vi "VF Laser Control.vi"(0 "Laser Notifier Element":T1={"Laser Action"=enum."Set On/Off", "Received?"=FALSE, "Enabled (Interlock)?"=FALSE, "Light Emission?"=FALSE, "Power (mW)"=0.0, "Settings"={"Laser Parameters"=enum."Wavelength (nm)", "Value"=0.0}, "Status"=enum."Error", "Error"={"status"=FALSE, "code"=0, "source"=""}}, 11 "VISA Ref":refnum<visa-resource-name>) -> (4 "Laser Notifier Element":T1={"Laser Action"=enum."Set On/Off", "Received?"=FALSE, "Enabled (Interlock)?"=FALSE, "Light Emission?"=FALSE, "Power (mW)"=0.0, "Settings"={"Laser Parameters"=enum."Wavelength (nm)", "Value"=0.0}, "Status"=enum."Error", "Error"={"status"=FALSE, "code"=0, "source"=""}})   [LabVIEW 2016]
uses:
  Laser Controls/Laser Notifier Element.ctl
  Laser Controls/Laser Actions.ctl
  Laser Controls/Laser Settings.ctl
  Laser Controls/Laser Parameters.ctl
  Laser Controls/Laser Status.ctl
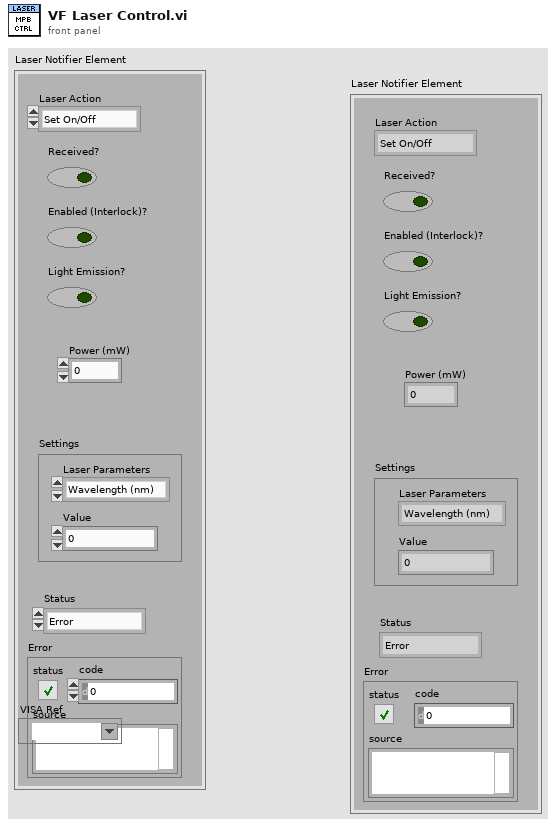
[diagram p1: front panel]
types:
  T1 = typedef "Laser Notifier Element.ctl" = cluster{"Laser Action":T2, "Received?":bool, "Enabled (Interlock)?":bool, "Light Emission?":bool, "Power (mW)":dbl, "Settings":T3, "Status":T5, "Error":errorcluster}
  T2 = typedef "Laser Actions.ctl" = enum16{"Error Check", "Set On/Off", "Set Power", "Set Parameter", "Get Power", "Get Status", "Get Parameter", "Quit"}
  T3 = typedef "Laser Settings.ctl" = cluster{"Laser Parameters":T4, "Value":dbl}
  T4 = typedef "Laser Parameters.ctl" = enum16{"Wavelength (nm)", "Pulsing?", "Rep. Rate"}
  T5 = typedef "Laser Status.ctl" = enum16{"Warmup", "Ready", "Emission", "Tuning", "Error"}
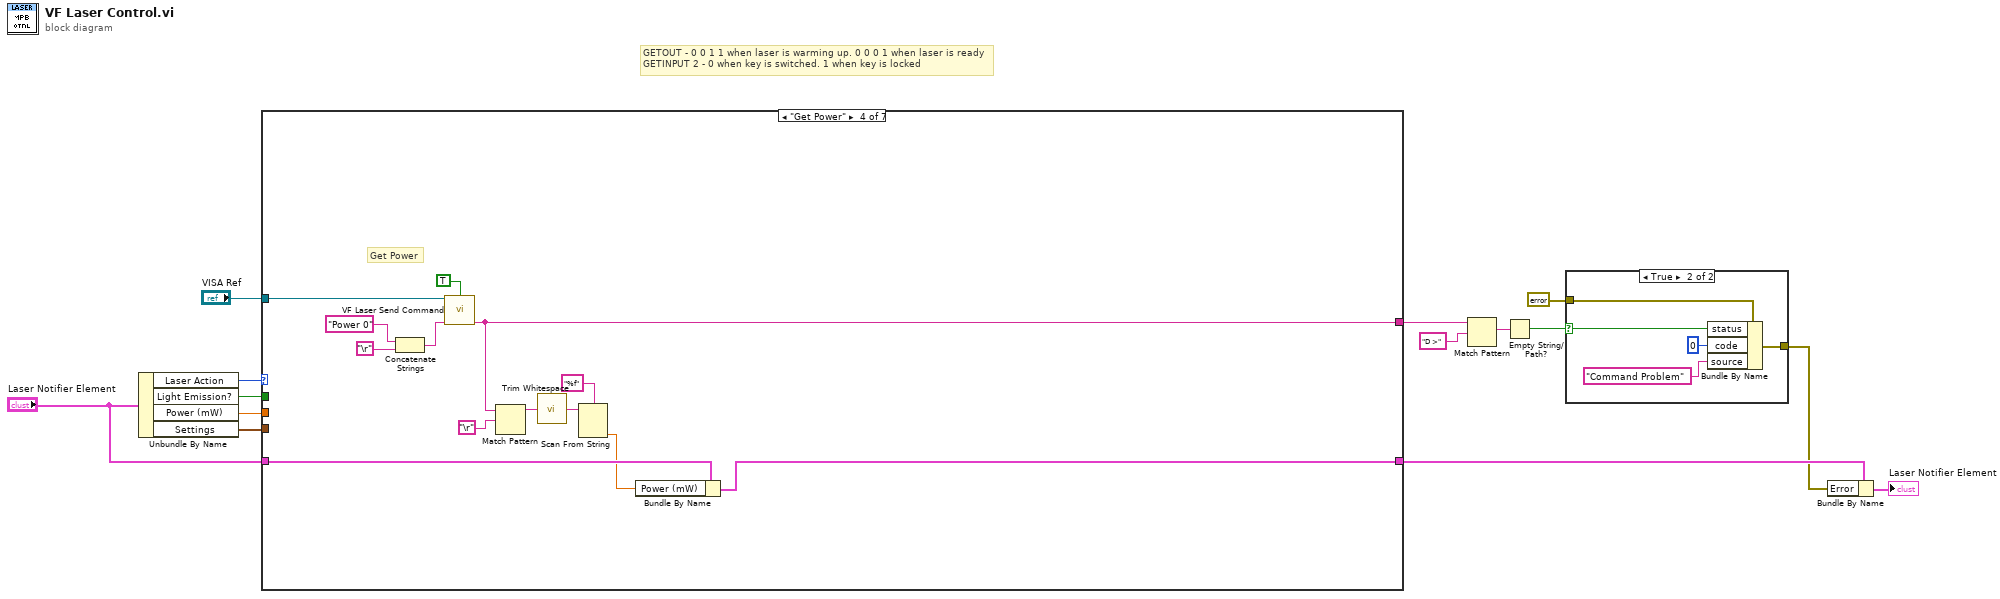
[diagram p0: block diagram]
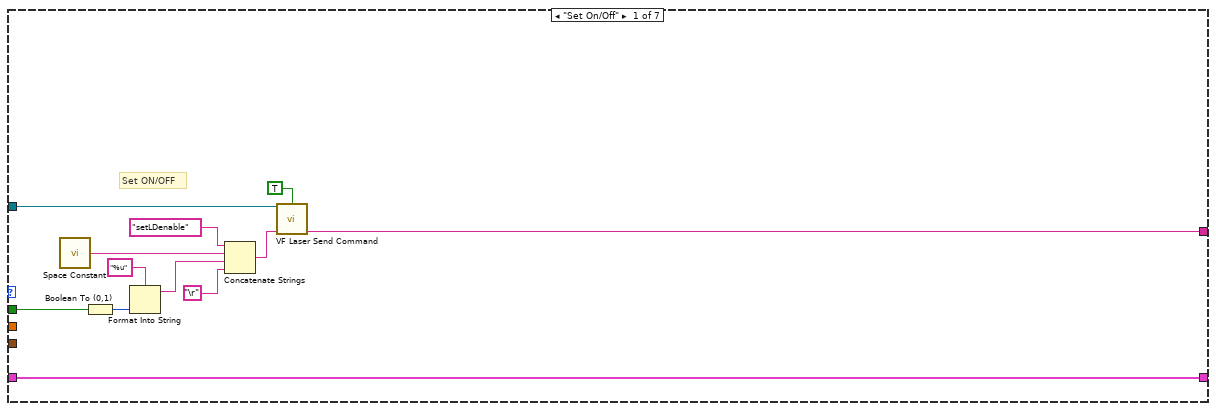
[diagram p3: hidden frame]
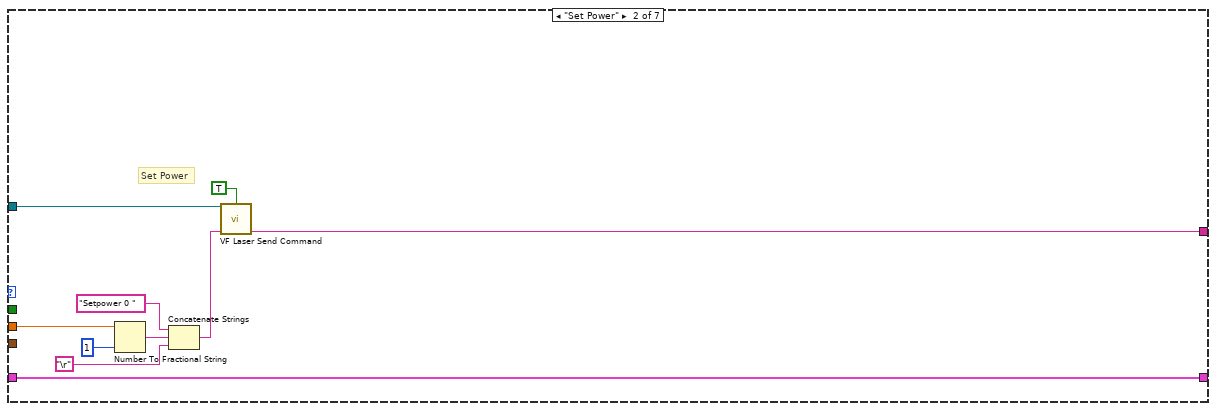
[diagram p4: hidden frame]
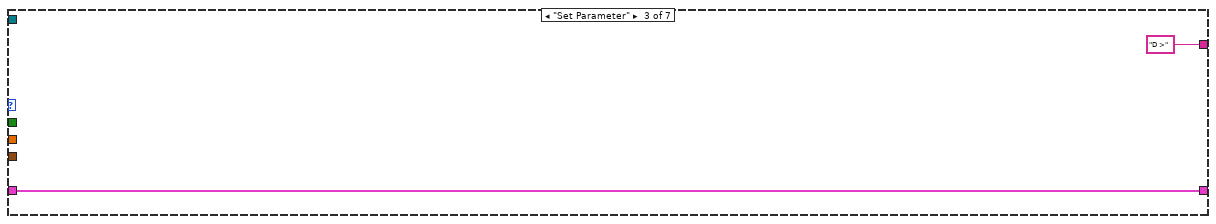
[diagram p5: hidden frame]
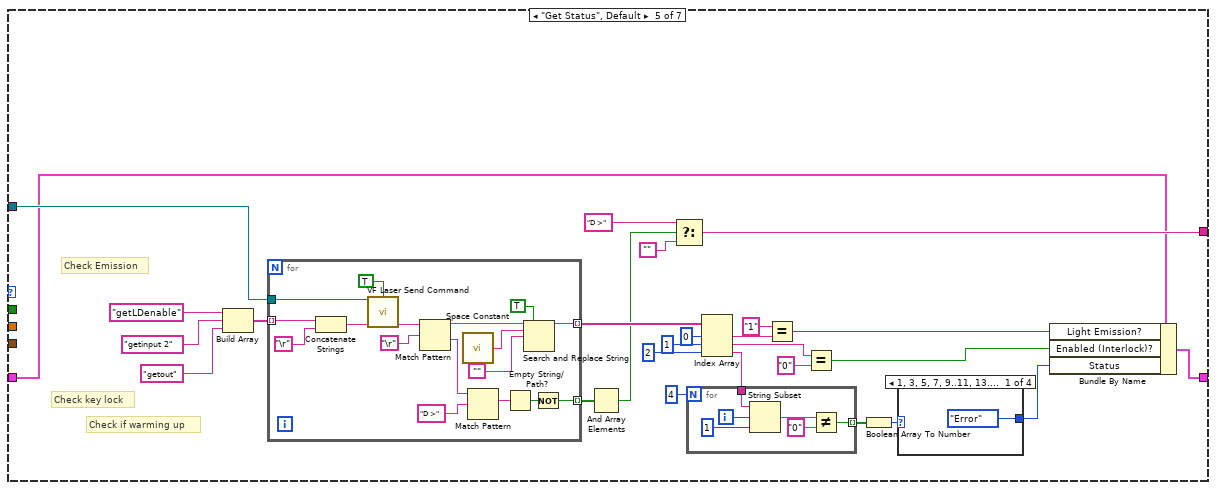
[diagram p6: hidden frame]
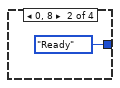
[diagram p7: hidden frame]
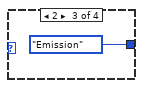
[diagram p8: hidden frame]
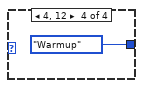
[diagram p9: hidden frame]
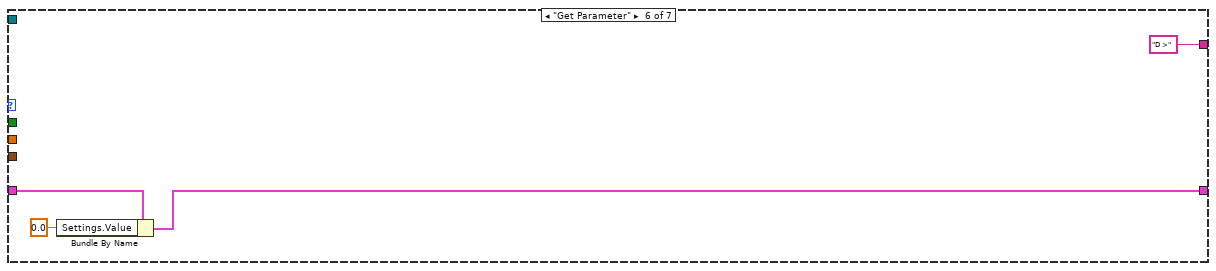
[diagram p10: hidden frame]
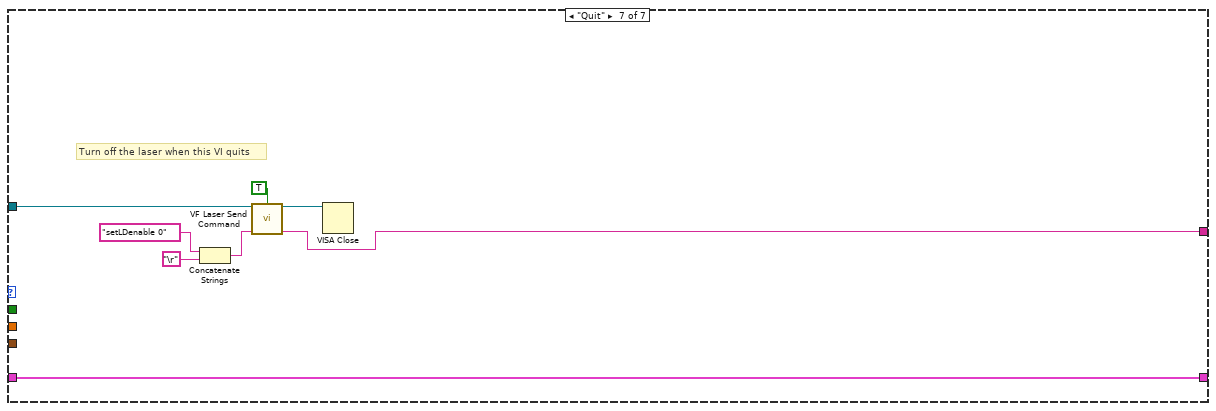
[diagram p11: hidden frame]
diagram:
  # "GETOUT - 0 0 1 1 when laser is warming up. 0 0 0 1 when laser is ready\nGETINPUT 2 - 0 when key is switched. 1 when key is locked"
  n1 = Unbundle By Name("Laser Notifier Element") -> ("Laser Action"=w14:T2, "Light Emission?"=w4:bool, "Power (mW)"=w3:dbl, "Settings"=w2:T3)
  n2 = case shown="\"Get Power\"" w14 {
    tunnel: "VISA Ref" -> [w18 w30 _ w43 w76 _ w111]
    tunnel: [w16 w28 "D >" ("Response") w42 w64 "D >" ("Response") w112] -> w12
    tunnel: [w15 w27 w38 w39 w75 w107 w110] -> w7
    tunnel: w4 -> [w17 _ _ _ _ _ _]
    tunnel: w3 -> [_ w29 _ _ _ _ _]
    tunnel: w2 -> [_ _ _ _ _ _ _]
    tunnel: "Laser Notifier Element" -> [w15 w27 w38 w41 w52 w109 w110]
    frame "Set On/Off" {
      # "Set ON/OFF"
      n3 = call <vilib>:"Space Constant.vi"() -> ("String"=w20:string)
      n4 = Boolean To (0,1)(Boolean=w17) -> (0, 1=w19:i16)
      n5 = Format Into String(format string="%u", w19) -> (resulting string=w22:string)  [unwired: 2 in, 1 out]
      n6 = Concatenate Strings("setLDenable" ("string"), w20, w22, "\r") -> (w25:string)
      n7 = call "VF Laser Send Command.vi"("VISA Ref"=w18, "Wait for Reply?"=TRUE, "Command"=w25) -> ("Response"=w16:string)  [unwired: 10 in, 2 out]
    }
    frame "Set Power" {
      # "Set Power"
      n8 = Number To Fractional String(number=w29, precision (6)=i16 1) -> (F-format string=w36:string)  [unwired: 2 in]
      n9 = Concatenate Strings("Setpower 0 " ("string"), w36, "\r") -> (w32:string)
      n10 = call "VF Laser Send Command.vi"("VISA Ref"=w30, "Wait for Reply?"=TRUE, "Command"=w32) -> ("Response"=w28:string)  [unwired: 10 in, 2 out]
    }
    frame "Set Parameter" {
    }
    frame "Get Power" {
      # "Get Power"
      n11 = Concatenate Strings("Power 0" ("string"), "\r") -> (w49:string)
      n12 = call "VF Laser Send Command.vi"("VISA Ref"=w43, "Wait for Reply?"=TRUE, "Command"=w49) -> ("Response"=w42:string)  [unwired: 10 in, 2 out]
      n13 = Match Pattern(string=w42, regular expression="\r") -> (before substring=w44:string)  [unwired: 1 in, 3 out]
      n14 = call <vilib>:"Trim Whitespace.vi"("string"=w44) -> ("trimmed string"=w46:string)  [unwired: 1 in]
      n15 = Scan From String(format string="%f", input string=w46) -> (output 1=w40:dbl)  [unwired: 3 in, 3 out]
      n16 = Bundle By Name(cluster=w41, "Power (mW)"=w40) -> (w39:T1)
    }
    frame "Get Status", Default {
      # "Check Emission"
      # "Check key lock"
      # "Check if warming up"
      n17 = Build Array("getLDenable" ("string"), "getinput 2" ("string"), "getout" ("string")) -> (w78:string[])
      n18 = for {
        tunnel: w78 -> [w102] mode=indexing
        tunnel: [w89] -> w72 mode=indexing
        tunnel: w76 -> [w101]
        tunnel: [w94] -> w68 mode=indexing
        n19 = Concatenate Strings(w102, "\r") -> (w104:string)
        n20 = call "VF Laser Send Command.vi"("VISA Ref"=w101, "Wait for Reply?"=TRUE, "Command"=w104) -> ("Response"=w99:string)  [unwired: 10 in, 2 out]
        n21 = Match Pattern(string=w99, regular expression="\r") -> (before substring=w90:string, after substring=w96:string)  [unwired: 1 in, 2 out]
        n22 = call <vilib>:"Space Constant.vi"() -> ("String"=w92:string)
        n23 = Match Pattern(string=w96, regular expression="D >" ("Response")) -> (match substring=w98:string)  [unwired: 1 in, 3 out]
        n24 = Empty String/Path?(string/path=w98) -> (empty?=w95:bool)
        n25 = Search and Replace String(replace all?=TRUE ("replace all? (F)"), input string=w90, search string=w92, replace string="") -> (result string=w89:string)  [unwired: 4 in, 3 out]
        n26 = Not(x=w95) -> (.not. x?=w94:bool)
      }
      n27 = And Array Elements(Boolean array=w68) -> (logical AND=w67:bool)
      n28 = Select(t="D >" ("Response"), s=w67, f="") -> (s? t:f=w64:string)
      n29 = Index Array(array=w72, index #1=0 ("index"), index #2=1 ("index"), index #3=2 ("index")) -> (element #1=w63:string, element #2=w58:string, element #3=w57:string)
      n30 = for {
        N: 4 -> [_]
        tunnel: [w84] -> w55 mode=indexing
        tunnel: w57 -> [w83]
        i -> [w87]
        n31 = String Subset(string=w83, offset (0)=w87, length (rest)=1 ("length (rest)")) -> (substring=w86:string)
        n32 = Not Equal?(x=w86, y="0") -> (x != y?=w84:bool)
      }
      n33 = Equal?(x="1", y=w63) -> (x = y?=w61:bool)
      n34 = Equal?(x=w58, y="0" ("x")) -> (x = y?=w59:bool)
      n35 = Boolean Array To Number(Boolean array=w55) -> (number=w54:u32)
      n36 = case shown="1, 3, 5, 7, 9..11, 13..15, Default" w54 {
        tunnel: [Laser_Status."Error" ("Status") Laser_Status."Ready" ("Status") Laser_Status."Emission" ("Status") Laser_Status."Warmup" ("Status")] -> w53
        frame 1, 3, 5, 7, 9..11, 13..15, Default {
        }
        frame 0, 8 {
        }
        frame 2 {
        }
        frame 4, 12 {
        }
      }
      n37 = Bundle By Name(cluster=w52, "Light Emission?"=w61, "Enabled (Interlock)?"=w59, "Status"=w53) -> (w75:T1)
    }
    frame "Get Parameter" {
      n38 = Bundle By Name(cluster=w109, "Settings.Value"=0.0) -> (w107:T1)
    }
    frame "Quit" {
      # "Turn off the laser when this VI quits"
      n39 = Concatenate Strings("setLDenable 0" ("string"), "\r") -> (w116:string)
      n40 = call "VF Laser Send Command.vi"("VISA Ref"=w111, "Wait for Reply?"=TRUE, "Command"=w116) -> ("VISA Ref Out"=w113:refnum<visa-resource-name>, "Response"=w112:string)  [unwired: 10 in, 1 out]
      n41 = VISA Close(VISA resource name=w113) -> ()  [unwired: 1 in, 1 out]
    }
  }
  n42 = Match Pattern(string=w12, regular expression="D >" ("Response")) -> (match substring=w10:string)  [unwired: 1 in, 3 out]
  n43 = Empty String/Path?(string/path=w10) -> (empty?=w9:bool)
  n44 = case shown="True" w9 {
    selector: w9 -> [_ w120]
    tunnel: errorcluster {"status"=FALSE, "code"=0, "source"=""} ("Error") -> [w118 w121]
    tunnel: [w118 w119] -> w5
    frame False {
    }
    frame True {
      n45 = Bundle By Name(cluster=w121, "status"=w120, "code"=0, "source"="Command Problem") -> (w119:errorcluster)
    }
  }
  n46 = Bundle By Name(cluster=w7, "Error"=w5) -> (→"Laser Notifier Element":T1)
